vi "Profile_Expand_Points.vi"(8 "error in (no error)":errorcluster={"status"=FALSE, "code"=0, "source"="\"\""}, 10 "configured axes":string, 11 "ProfileDefinition":string) -> (0 "error out":errorcluster={"status"=FALSE, "code"=0, "source"="\"\""}, 2 "status ok":bool, 3 "Ordered operating-point list":string)   [LabVIEW 2026]
doc: "INTENT: Expand generic operating-point sweep. LOGIC: Generate pressure-only, flow-only, combined or explicit table points respecting configured order."
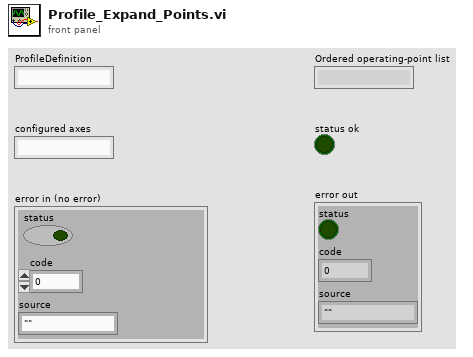
[diagram p1: front panel]
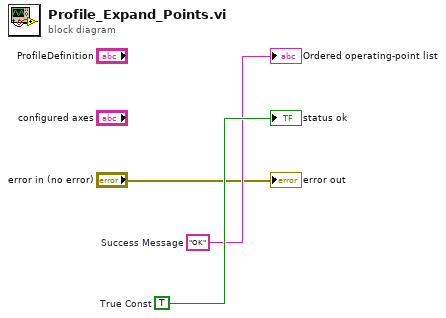
[diagram p0: block diagram]
diagram:
  w3 = TRUE  # True Const
  w2 = "OK"  # Success Message
  "Ordered operating-point list" <- w2
  "status ok" <- w3
  "error out" <- "error in (no error)"
